vi "Main UI.vi"(8 "error in (no error)":errorcluster, 11 "picoG in":refnum<class "picoG.lvclass">) -> (0 "error out":errorcluster, 3 "picoG out":refnum<class "picoG.lvclass">)   [LabVIEW 2020, in "PicoG-App.lvlib" / "picoG.lvclass"]
uses:
  picoG.lvclass
  UI State.ctl
  picoG.lvclass/picoG.ctl
  AppListPanel/AppListPanel.lvclass
  C:/Program Files (x86)/National Instruments/LabVIEW 2020/vi.lib/IlluminatedG/IG OOPanel/OOPanel/Panel/Panel.lvclass
  DeviceListPanel/DeviceListPanel.lvclass
  GettingStarted/GettingStarted.lvclass
  PlatformListPanel/PlatformListPanel.lvclass
  AppDetailPanel/AppDetailPanel.lvclass
  DeviceDetailPanel/DeviceDetailPanel.lvclass
  PlatformConfigPanel/PlatformConfigPanel.lvclass
  AppListPanel/Panel.vi
  ViaApp/ViaApp.lvclass
  Builds/picoG/ppl/PicoG-Core.lvlibp/PicoG-Processor/PicoG-Core/Platform/Platform.lvclass
  Device/Device.lvclass
  <vilib>/IlluminatedG/IG OOPanel/OOPanel/Manager/Manager.lvclass
  PicoG-App.lvlib
  App Watcher/App Watcher.lvclass
panel:
  in  "System":bool
  in  "Devices":bool
  in  "Apps":bool
  in  "Platforms":bool
  in  "OK Button":bool
  out "StatusLeft":string
  out "StatusLeft 2":string
  out "StatusRight 2":string
  out "ProgressBar":dbl(slide) scale=0.0..100.0
  out "StatusRight":string
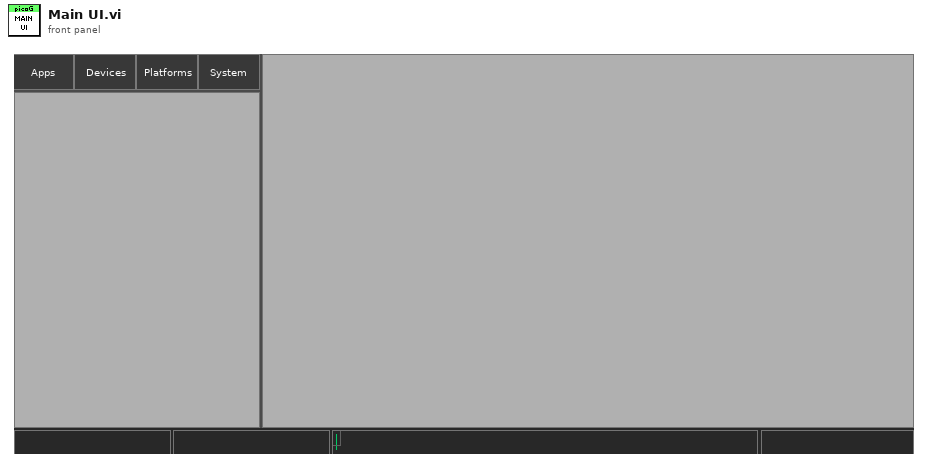
[diagram p1: front panel]
types:
  T1 = typedef "PicoG-App.lvlib/picoG.lvclass/UI State.ctl" = enum16{"Init", "Run", "Close"}
  T2 = enum32{"Invalid", "Standard", "Closed", "Hidden", "Minimized", "Maximized"}
  T3 = typedef "PicoG-App.lvlib/picoG.lvclass/Inbound Events.ctl" = cluster{"Add App":refnum<user-event>, "App Update":refnum<user-event>, "Select App":refnum<user-event>, "Select Platform":refnum<user-event>, "Add Device":refnum<user-event>, "Select Device":refnum<user-event>, "Remove App":refnum<user-event>, "Deploy Event":refnum<user-event>, "Remove Device":refnum<user-event>, "Refresh Device":refnum<user-event>}
  T4 = typedef "PicoG-App.lvlib/Device.lvclass/Device Key.ctl" = cluster{"Platform":string, "Board":string, "ID":string}
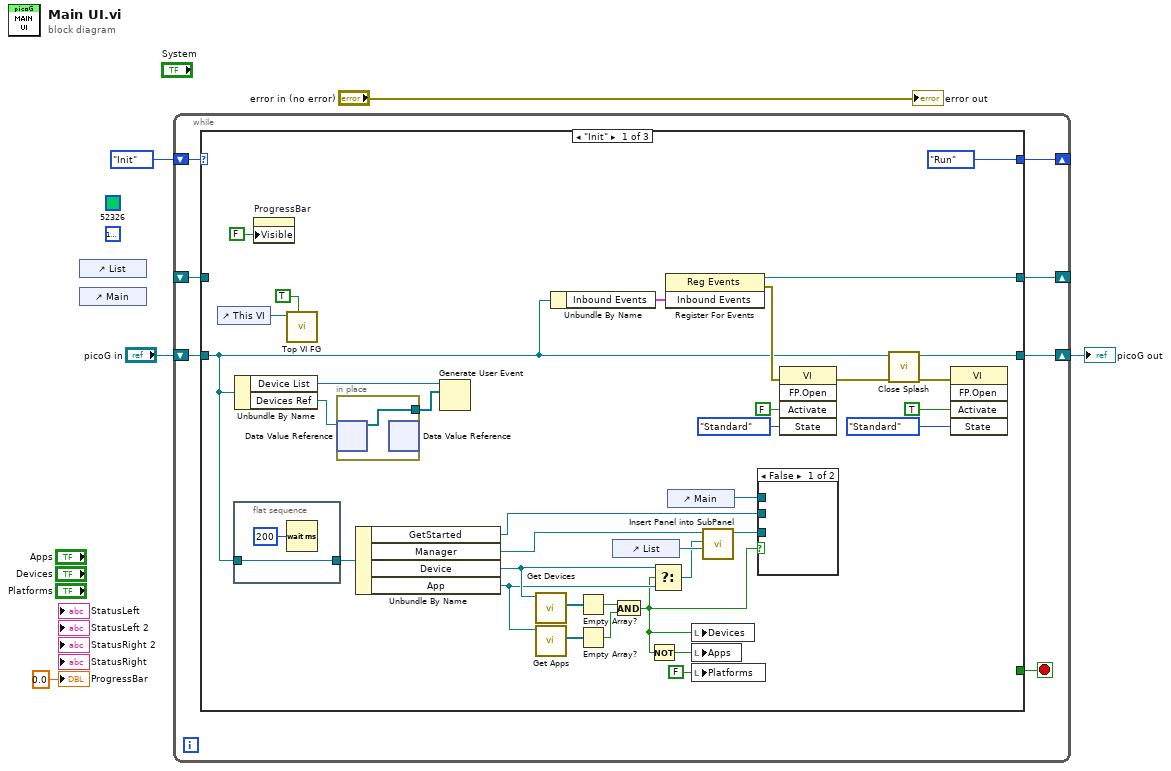
[diagram p0: block diagram]
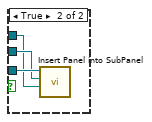
[diagram p2: hidden frame]
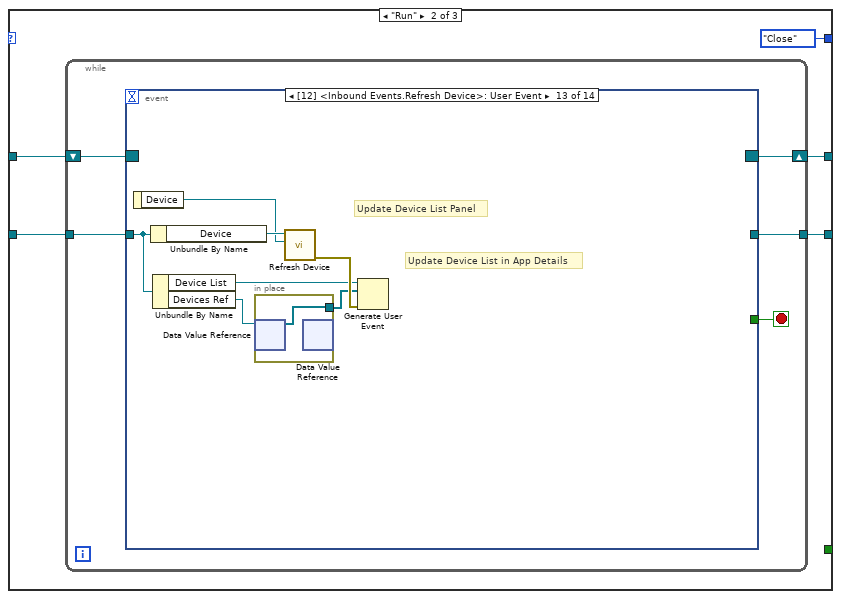
[diagram p3: hidden frame]
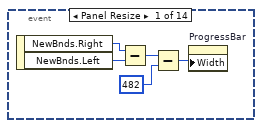
[diagram p4: hidden frame]
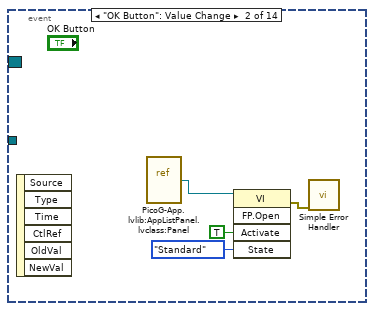
[diagram p5: hidden frame]
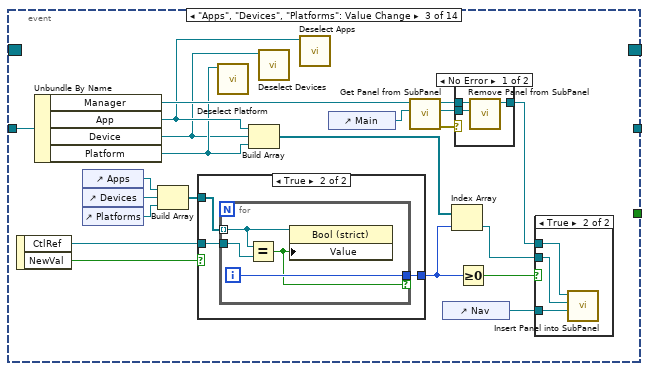
[diagram p6: hidden frame]
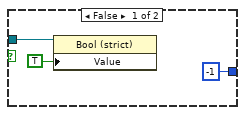
[diagram p9: hidden frame]
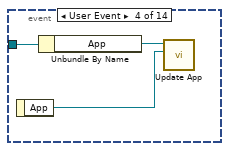
[diagram p10: hidden frame]
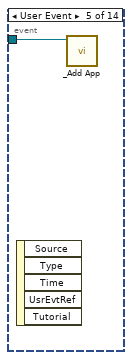
[diagram p11: hidden frame]
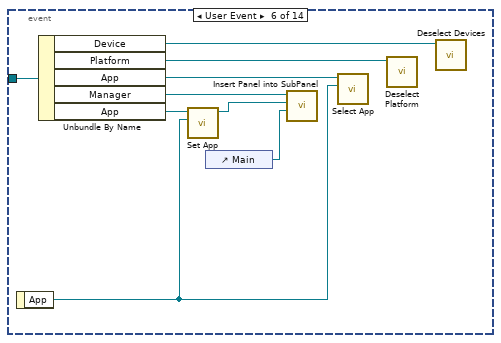
[diagram p12: hidden frame]
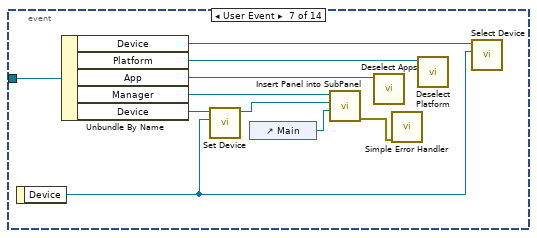
[diagram p13: hidden frame]
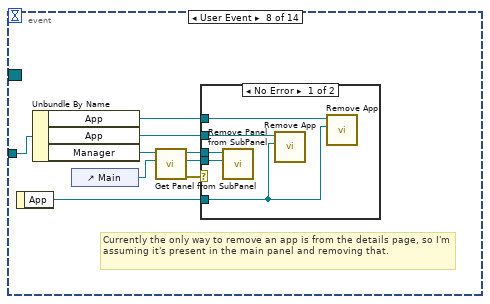
[diagram p14: hidden frame]
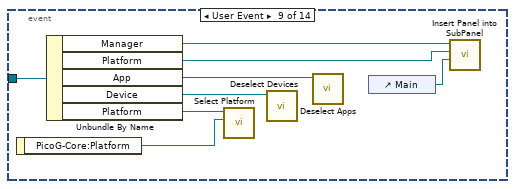
[diagram p16: hidden frame]
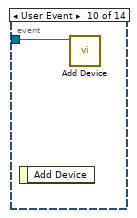
[diagram p17: hidden frame]
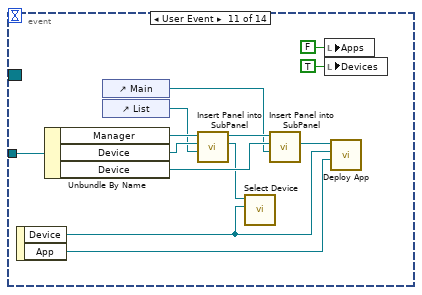
[diagram p18: hidden frame]
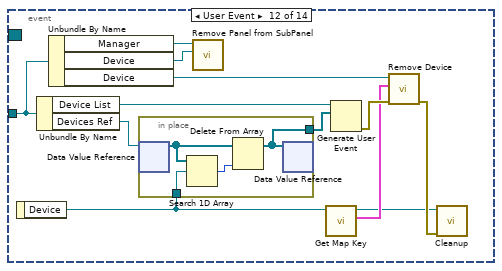
[diagram p19: hidden frame]
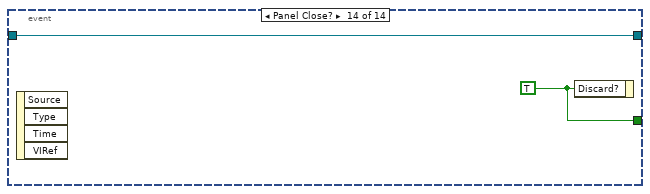
[diagram p20: hidden frame]
diagram:
  (unwired) u32 16777216
  (unwired) u32 52326
  n1 = control-ref of="List"() -> ()  [unwired: 1 out]
  n2 = control-ref of="Main"() -> ()  [unwired: 1 out]
  n3 = while {
    shift-right: [w11] -> _
    shift-left: UI_State."Init" ("UI State") -> [w12]
    shift-right: [w8] -> w2
    shift-left: "picoG in" -> [w9]
    shift-right: [w7] -> _
    shift-left: _ -> [w6]
    stop <- w10 stop-if-true
    n4 = case shown="\"Init\"" w12 {
      selector: w12 -> [_ _ w201]
      tunnel: [UI_State."Run" ("UI State") UI_State."Close" ("UI State") w201] -> w11
      tunnel: [_ _ TRUE] -> w10
      tunnel: w9 -> [w14 w56 w197]
      tunnel: [w38 w55 w196] -> w8
      tunnel: [w35 w53 _] -> w7
      tunnel: w6 -> [_ w54 w198]
      frame "Init" {
        n5 = control-ref of="This VI"() -> (w34:refnum<vi>)
        n6 = flat-sequence {
          tunnel: w14 -> [w49]
          tunnel: [w49] -> w18
          frame #0 {
            n7 = Wait (ms)(milliseconds to wait=u32 200) -> ()  [unwired: 1 out]
          }
        }
        n8 = Unbundle By Name(w14) -> ("Device List"=w16:refnum<user-event>, "Devices Ref"=w17:refnum<data-value>)
        n9 = property on="ProgressBar" class="Slide (strict)"("Visible"=FALSE) -> ()  [unwired: 2 in, 2 out]
        n10 = call "Top VI FG.vi"("Set (F)"=TRUE, "Top-Level VI In"=w34) -> ()  [unwired: 8 in, 2 out]
        n11 = in-place {
          in-place-border: [w47] -> w15
          n12 = in-place-dvr #1(w17) -> (w47:refnum<class "Device.lvclass">[])  [unwired: 1 out]
          n13 = in-place-dvr #1() -> ()  [unwired: 1 in, 2 out]
        }
        n14 = Unbundle By Name(w18) -> ("GetStarted"=w21:refnum<class "GettingStarted.lvclass">, "Manager"=w24:refnum<class "Manager.lvclass">, "Device"=w27:refnum<class "DeviceListPanel.lvclass">, "App"=w26:refnum<class "AppListPanel.lvclass">)
        n15 = Generate User Event(user event=w16, event data cluster=w15) -> ()  [unwired: 2 in, 2 out]
        n16 = call "Get Devices.vi"("DeviceListPanel in"=w27) -> ("Devices"=w30:refnum<class "Device.lvclass">[])  [unwired: 8 in, 2 out]
        n17 = call "Get Apps.vi"("AppListPanel in"=w26) -> ("Apps"=w31:refnum<class "ViaApp.lvclass">[])  [unwired: 8 in, 2 out]
        n18 = Unbundle By Name(w14) -> ("Inbound Events"=w36:T3)
        n19 = Empty Array?(array=w30) -> (empty?=w28:bool)
        n20 = Empty Array?(array=w31) -> (empty?=w29:bool)
        n21 = control-ref of="List"() -> (w37:refnum<vi>)
        n22 = And(x=w28, y=w29) -> (x .and. y?=w19:bool)
        n23 = Not(x=w19) -> (.not. x?=w20:bool)
        n24 = Select(t=w27, s=w19, f=w26) -> (s? t:f=w25:refnum<class "Panel.lvclass">)
        n25 = register-events(w36) -> (reference out=w35:refnum<event-registration>, error out=w46:errorcluster)  [unwired: 2 in]
        n26 = control-ref of="Main"() -> (w23:refnum<vi>)
        n27 = local write "Devices"(w19) -> ()
        n28 = local write "Apps"(w20) -> ()
        n29 = local write "Platforms"(FALSE ("Nav Devices")) -> ()
        n30 = call <vilib>:"Insert Panel into SubPanel.vi"("SubPanel"=w37, "Panel In"=w25, "Manager in"=w24) -> ("Manager out"=w22:refnum<class "Manager.lvclass">)  [unwired: 6 in, 2 out]
        n31 = case shown="False" w19 {
          tunnel: w23 -> [_ w50]
          tunnel: w22 -> [_ w52]
          tunnel: w21 -> [_ w51]
          frame False {
          }
          frame True {
            n32 = call <vilib>:"Insert Panel into SubPanel.vi"("SubPanel"=w50, "Panel In"=w51, "Manager in"=w52) -> ()  [unwired: 6 in, 3 out]
          }
        }
        n33 = invoke class="VI" method="FP.Open"(error in=w46, "Activate"=FALSE ("Activate?"), "State"=T2."Standard") -> (error out=w42:errorcluster)  [unwired: 2 in, 4 out]
        n34 = call "Close Splash.vi"("error in (no error)"=w42, "picoG in"=w14) -> ("error out"=w41:errorcluster, "picoG out"=w38:refnum<class "picoG.lvclass">)  [unwired: 8 in]
        n35 = invoke class="VI" method="FP.Open"(error in=w41, "Activate"=TRUE ("Activate?"), "State"=T2."Standard") -> ()  [unwired: 2 in, 5 out]
      }
      frame "Run" {
        n36 = while {
          tunnel: w56 -> [w61]
          tunnel: [w60] -> w55
          shift-right: [w58] -> w53
          shift-left: w54 -> [w59]
          stop <- w62 stop-if-true
          n37 = event shown="[12] <Inbound Events.Refresh Device>: User Event" {
            selector: w59 -> [_ _ _ _ _ _ _ _ _ _ _ _ _ _]
            dyn-events: [_ _ _ _ _ _ _ _ _ _ _ _ _ _] -> w58
            timeout: _ -> [_ _ _ _ _ _ _ _ _ _ _ _ _ _]
            tunnel: [_ _ _ _ _ _ _ _ _ _ _ _ _ w194] -> w62
            tunnel: w61 -> [_ _ w83 w112 w113 w122 w130 w141 w154 w155 w168 w177 w188 w193]
            tunnel: [_ _ _ _ _ _ _ _ _ _ _ _ _ w193] -> w60
            event Panel Resize {
              n38 = event-data() -> ("NewBnds.Right"=w66:i16, "NewBnds.Left"=w67:i16)  [unwired: 1 in]
              n39 = Subtract(x=w66, y=w67) -> (x-y=w65:i16)
              n40 = Subtract(x=w65, y=i16 482) -> (x-y=w63:i16)
              n41 = property on="ProgressBar" class="Slide (strict)"("Width"=w63) -> ()  [unwired: 2 in, 2 out]
            }
            event "OK Button": Value Change {
              n42 = event-data() -> ()  [unwired: 1 in, 6 out]
              n43 = vi-ref "PicoG-App.lvlib:AppListPanel.lvclass:Panel.vi"() -> (w71:refnum<vi>)
              n44 = invoke class="VI" method="FP.Open"(reference=w71, "Activate"=TRUE ("Activate?"), "State"=T2."Standard") -> (error out=w68:errorcluster)  [unwired: 2 in, 4 out]
              n45 = call <vilib>:"Simple Error Handler.vi"("error in (no error)"=w68) -> ()  [unwired: 4 in, 5 out]
            }
            event "Apps", "Devices", "Platforms": Value Change {
              n46 = event-data() -> ("CtlRef"=w91:refnum<vi>, "NewVal"=w92:bool)  [unwired: 1 in]
              n47 = Unbundle By Name(w83) -> ("Manager"=w80:refnum<class "Manager.lvclass">, "App"=w75:refnum<class "AppListPanel.lvclass">, "Device"=w72:refnum<class "DeviceListPanel.lvclass">, "Platform"=w74:refnum<class "PlatformListPanel.lvclass">)
              n48 = control-ref of="Apps"() -> (w89:refnum<vi>)
              n49 = control-ref of="Devices"() -> (w90:refnum<vi>)
              n50 = control-ref of="Platforms"() -> (w88:refnum<vi>)
              n51 = Build Array(w89, w90, w88) -> (w81:refnum<vi>[])
              n52 = case shown="True" w92 {
                tunnel: w91 -> [w102 w105]
                tunnel: w81 -> [_ w104]
                tunnel: [-1 w103] -> w87
                frame False {
                  n53 = property class="Bool (strict)"(reference=w102, "Value"=TRUE) -> ()  [unwired: 1 in, 2 out]
                }
                frame True {
                  n54 = for {
                    tunnel: w105 -> [w109]
                    tunnel: w104 -> [w108] mode=indexing
                    tunnel: [w107] -> w103 if=w106
                    i -> [w107]
                    n55 = Equal?(x=w108, y=w109) -> (x = y?=w106:bool)
                    n56 = property class="Bool (strict)"(reference=w108, "Value"=w106) -> ()  [unwired: 1 in, 2 out]
                  }
                }
              }
              n57 = call "Deselect Platform.vi"("PlatformListPanel in"=w74) -> ()  [unwired: 9 in, 2 out]
              n58 = Build Array(w75, w72, w74) -> (w82:refnum<class "Panel.lvclass">[])
              n59 = call "Deselect Devices.vi"("DeviceListPanel in"=w72) -> ()  [unwired: 9 in, 2 out]
              n60 = call "Deselect Apps.vi"("AppListPanel in"=w75) -> ()  [unwired: 9 in, 2 out]
              n61 = control-ref of="Main"() -> (w79:refnum<vi>)
              n62 = call <vilib>:"Get Panel from SubPanel.vi"("SubPanel"=w79, "Manager in"=w80) -> ("error out"=w73:errorcluster, "Panel"=w77:refnum<class "Panel.lvclass">, "Manager out"=w78:refnum<class "Manager.lvclass">)  [unwired: 7 in]
              n63 = control-ref of="Nav"() -> (w85:refnum<vi>)
              n64 = Index Array(array=w82, index=w87) -> (element=w84:refnum<class "Panel.lvclass">)
              n65 = case shown="No Error" w73 {
                tunnel: w78 -> [w95 w96]
                tunnel: w77 -> [w94 _]
                tunnel: [w93 w96] -> w76
                frame No Error {
                  n66 = call <vilib>:"Remove Panel from SubPanel.vi"("Panel In"=w94, "Manager in"=w95) -> ("Manager out"=w93:refnum<class "Manager.lvclass">)  [unwired: 7 in, 2 out]
                }
                frame Error {
                }
              }
              n67 = Greater Or Equal To 0?(x=w87) -> (x >= 0?=w86:bool)
              n68 = case shown="True" w86 {
                tunnel: w85 -> [_ w99]
                tunnel: w84 -> [_ w98]
                tunnel: w76 -> [_ w97]
                frame False {
                }
                frame True {
                  n69 = call <vilib>:"Insert Panel into SubPanel.vi"("SubPanel"=w99, "Panel In"=w98, "Manager in"=w97) -> ()  [unwired: 6 in, 3 out]
                }
              }
            }
            event User Event {
              n70 = event-data() -> ("App"=w110:refnum<class "ViaApp.lvclass">)  [unwired: 1 in]
              n71 = Unbundle By Name(w112) -> ("App"=w111:refnum<class "AppListPanel.lvclass">)
              n72 = call "Update App.vi"("ViaApp"=w110, "AppListPanel in"=w111) -> ()  [unwired: 8 in, 2 out]
            }
            event User Event {
              n73 = event-data() -> ()  [unwired: 1 in, 5 out]
              n74 = call "_Add App.vi"("picoG in"=w113) -> ()  [unwired: 9 in, 2 out]
            }
            event User Event {
              n75 = event-data() -> ("App"=w118:refnum<class "ViaApp.lvclass">)  [unwired: 1 in]
              n76 = Unbundle By Name(w122) -> ("Device"=w114:refnum<class "DeviceListPanel.lvclass">, "Platform"=w120:refnum<class "PlatformListPanel.lvclass">, "App"=w121:refnum<class "AppListPanel.lvclass">, "Manager"=w117:refnum<class "Manager.lvclass">, "App"=w119:refnum<class "AppDetailPanel.lvclass">)
              n77 = call "Set App.vi"("App"=w118, "AppDetailPanel in"=w119) -> ("AppDetailPanel out"=w115:refnum<class "AppDetailPanel.lvclass">)  [unwired: 8 in, 1 out]
              n78 = control-ref of="Main"() -> (w116:refnum<vi>)
              n79 = call <vilib>:"Insert Panel into SubPanel.vi"("SubPanel"=w116, "Panel In"=w115, "Manager in"=w117) -> ()  [unwired: 6 in, 3 out]
              n80 = call "Select App.vi"("App"=w118, "AppListPanel in"=w121) -> ()  [unwired: 8 in, 2 out]
              n81 = call "Deselect Platform.vi"("PlatformListPanel in"=w120) -> ()  [unwired: 9 in, 2 out]
              n82 = call "Deselect Devices.vi"("DeviceListPanel in"=w114) -> ()  [unwired: 9 in, 2 out]
            }
            event User Event {
              n83 = event-data() -> ("Device"=w126:refnum<class "Device.lvclass">)  [unwired: 1 in]
              n84 = Unbundle By Name(w130) -> ("Device"=w129:refnum<class "DeviceListPanel.lvclass">, "Platform"=w132:refnum<class "PlatformListPanel.lvclass">, "App"=w125:refnum<class "AppListPanel.lvclass">, "Manager"=w131:refnum<class "Manager.lvclass">, "Device"=w128:refnum<class "DeviceDetailPanel.lvclass">)
              n85 = call "Set Device.vi"("Device"=w126, "DeviceDetailPanel in"=w128) -> ("DeviceDetailPanel out"=w127:refnum<class "DeviceDetailPanel.lvclass">)  [unwired: 8 in, 1 out]
              n86 = control-ref of="Main"() -> (w123:refnum<vi>)
              n87 = call <vilib>:"Insert Panel into SubPanel.vi"("SubPanel"=w123, "Panel In"=w127, "Manager in"=w131) -> ("error out"=w124:errorcluster)  [unwired: 6 in, 2 out]
              n88 = call "Deselect Apps.vi"("AppListPanel in"=w125) -> ()  [unwired: 9 in, 2 out]
              n89 = call <vilib>:"Simple Error Handler.vi"("error in (no error)"=w124) -> ()  [unwired: 4 in, 5 out]
              n90 = call "Deselect Platform.vi"("PlatformListPanel in"=w132) -> ()  [unwired: 9 in, 2 out]
              n91 = call "Select Device.vi"("Device"=w126, "DeviceListPanel in"=w129) -> ()  [unwired: 8 in, 2 out]
            }
            event User Event {
              # "Currently the only way to remove an app is from the details page, so I'm assuming it's present in the main panel and removing that."
              n92 = event-data() -> ("App"=w136:refnum<class "ViaApp.lvclass">)  [unwired: 1 in]
              n93 = Unbundle By Name(w141) -> ("App"=w133:refnum<class "App Watcher.lvclass">, "App"=w134:refnum<class "AppListPanel.lvclass">, "Manager"=w140:refnum<class "Manager.lvclass">)
              n94 = control-ref of="Main"() -> (w139:refnum<vi>)
              n95 = call <vilib>:"Get Panel from SubPanel.vi"("SubPanel"=w139, "Manager in"=w140) -> ("error out"=w137:errorcluster, "Panel"=w138:refnum<class "Panel.lvclass">, "Manager out"=w135:refnum<class "Manager.lvclass">)  [unwired: 7 in]
              n96 = case shown="No Error" w137 {
                tunnel: w138 -> [w146 _]
                tunnel: w136 -> [w142 _]
                tunnel: w135 -> [w145 _]
                tunnel: w134 -> [w144 _]
                tunnel: w133 -> [w143 _]
                frame No Error {
                  n97 = call <vilib>:"Remove Panel from SubPanel.vi"("Panel In"=w146, "Manager in"=w145) -> ()  [unwired: 7 in, 3 out]
                  n98 = call "Remove App.vi"("App"=w142, "AppListPanel in"=w144) -> ()  [unwired: 8 in, 2 out]
                  n99 = call "Remove App.vi"("App"=w142, "App Watcher in"=w143) -> ()  [unwired: 8 in, 2 out]
                }
                frame Error {
                  # "#ERROR?"
                }
              }
            }
            event User Event {
              n100 = event-data() -> ("PicoG-Core:Platform"=w152:refnum<class "Platform.lvclass">)  [unwired: 1 in]
              n101 = Unbundle By Name(w154) -> ("Manager"=w149:refnum<class "Manager.lvclass">, "Platform"=w148:refnum<class "PlatformConfigPanel.lvclass">, "App"=w151:refnum<class "AppListPanel.lvclass">, "Device"=w147:refnum<class "DeviceListPanel.lvclass">, "Platform"=w153:refnum<class "PlatformListPanel.lvclass">)
              n102 = call "Select Platform.vi"("Platform"=w152, "PlatformListPanel in"=w153) -> ()  [unwired: 8 in, 2 out]
              n103 = call "Deselect Devices.vi"("DeviceListPanel in"=w147) -> ()  [unwired: 9 in, 2 out]
              n104 = call "Deselect Apps.vi"("AppListPanel in"=w151) -> ()  [unwired: 9 in, 2 out]
              n105 = control-ref of="Main"() -> (w150:refnum<vi>)
              n106 = call <vilib>:"Insert Panel into SubPanel.vi"("SubPanel"=w150, "Panel In"=w148, "Manager in"=w149) -> ()  [unwired: 6 in, 3 out]
            }
            event User Event {
              n107 = event-data() -> ()  [unwired: 1 in, 1 out]
              n108 = call "Add Device.vi"("picoG in"=w155) -> ()  [unwired: 9 in, 2 out]
            }
            event User Event {
              n109 = event-data() -> ("Device"=w159:refnum<class "Device.lvclass">, "App"=w158:refnum<class "ViaApp.lvclass">)  [unwired: 1 in]
              n110 = Unbundle By Name(w168) -> ("Manager"=w167:refnum<class "Manager.lvclass">, "Device"=w166:refnum<class "DeviceListPanel.lvclass">, "Device"=w164:refnum<class "DeviceDetailPanel.lvclass">)
              n111 = control-ref of="Main"() -> (w156:refnum<vi>)
              n112 = control-ref of="List"() -> (w157:refnum<vi>)
              n113 = call <vilib>:"Insert Panel into SubPanel.vi"("SubPanel"=w157, "Panel In"=w166, "Manager in"=w167) -> ("Panel"=w161:refnum<class "DeviceListPanel.lvclass">, "Manager out"=w165:refnum<class "Manager.lvclass">)  [unwired: 6 in, 1 out]
              n114 = call "Select Device.vi"("Device"=w159, "DeviceListPanel in"=w161) -> ()  [unwired: 8 in, 2 out]
              n115 = call <vilib>:"Insert Panel into SubPanel.vi"("SubPanel"=w156, "Panel In"=w164, "Manager in"=w165) -> ("Panel"=w160:refnum<class "DeviceDetailPanel.lvclass">)  [unwired: 6 in, 2 out]
              n116 = local write "Apps"(FALSE ("Apps")) -> ()
              n117 = local write "Devices"(TRUE ("Devices")) -> ()
              n118 = call "Deploy App.vi"("App"=w158, "Device"=w159, "DeviceDetailPanel in"=w160) -> ()  [unwired: 7 in, 2 out]
            }
            event User Event {
              n119 = event-data() -> ("Device"=w171:refnum<class "Device.lvclass">)  [unwired: 1 in]
              n120 = Unbundle By Name(w177) -> ("Device List"=w179:refnum<user-event>, "Devices Ref"=w180:refnum<data-value>)
              n121 = Unbundle By Name(w177) -> ("Manager"=w173:refnum<class "Manager.lvclass">, "Device"=w172:refnum<class "DeviceDetailPanel.lvclass">, "Device"=w176:refnum<class "DeviceListPanel.lvclass">)
              n122 = in-place {
                in-place-border: w171 -> [w184]
                in-place-border: [w181] -> w178
                n123 = in-place-dvr #2(w180) -> (w183:refnum<class "Device.lvclass">[])  [unwired: 1 out]
                n124 = Search 1D Array(1D array=w183, element=w184) -> (index of element=w182:i32)  [unwired: 1 in]
                n125 = Delete From Array(array=w183, index=w182) -> (array with subset deleted=w181:refnum<class "Device.lvclass">[])  [unwired: 1 in, 1 out]
                n126 = in-place-dvr #2(w181) -> ()  [unwired: 2 out]
              }
              n127 = call <vilib>:"Remove Panel from SubPanel.vi"("Panel In"=w172, "Manager in"=w173) -> ()  [unwired: 7 in, 3 out]
              n128 = call "Get Map Key.vi"("Device in"=w171) -> ("Key"=w170:T4, "Device out"=w169:refnum<class "Device.lvclass">)  [unwired: 8 in, 1 out]
              n129 = Generate User Event(user event=w179, event data cluster=w178) -> (error out=w175:errorcluster)  [unwired: 2 in, 1 out]
              n130 = call "Remove Device.vi"("error in (no error)"=w175, "Key"=w170, "DeviceListPanel in"=w176) -> ("error out"=w174:errorcluster)  [unwired: 7 in, 1 out]
              n131 = call "Cleanup.vi"("error in (no error)"=w174, "Device in"=w169) -> ()  [unwired: 9 in, 1 out]
            }
            event User Event {
              # "Update Device List in App Details"
              # "Update Device List Panel"
              n132 = event-data() -> ("Device"=w189:refnum<class "Device.lvclass">)  [unwired: 1 in]
              n133 = Unbundle By Name(w188) -> ("Device"=w190:refnum<class "DeviceListPanel.lvclass">)
              n134 = Unbundle By Name(w188) -> ("Device List"=w185:refnum<user-event>, "Devices Ref"=w187:refnum<data-value>)
              n135 = in-place {
                in-place-border: [w192] -> w186
                n136 = in-place-dvr #3(w187) -> (w192:refnum<class "Device.lvclass">[])  [unwired: 1 out]
                n137 = in-place-dvr #3() -> ()  [unwired: 1 in, 2 out]
              }
              n138 = call "Refresh Device.vi"("Device"=w189, "DeviceListPanel in"=w190) -> ("error out"=w191:errorcluster)  [unwired: 8 in, 1 out]
              n139 = Generate User Event(user event=w185, event data cluster=w186, error in=w191) -> ()  [unwired: 1 in, 2 out]
            }
            event Panel Close? {
              w194 = TRUE ("Discard?")
              n140 = event-data() -> ()  [unwired: 1 in, 4 out]
              n141 = event-data("Discard?"=w194) -> ()  [unwired: 1 in, 1 out]
            }
          }
        }
      }
      frame "Close" {
        # "Save configs here before everything gets cleaned up in... Cleanup.vi"
        n142 = Unregister For Events(event registration refnum=w198) -> ()  [unwired: 1 in, 1 out]
        n143 = call "Save Config.vi"("picoG in"=w197) -> ("error out"=w195:errorcluster, "picoG out"=w196:refnum<class "picoG.lvclass">)  [unwired: 9 in]
        n144 = call <vilib>:"Simple Error Handler.vi"("error in (no error)"=w195) -> ()  [unwired: 4 in, 5 out]
        n145 = control-ref of="This VI"() -> (w199:refnum<vi>)
        n146 = invoke class="VI" method="FP.Close"(reference=w199) -> ()  [unwired: 2 in, 3 out]
      }
    }
  }
  "picoG out" <- w2
  "error out" <- "error in (no error)"
  "ProgressBar" <- 0.0 ("ProgressBar")
